vi "output.vi"(8 "error in":errorcluster, 10 "data table in":T1, 11 "Modbus Slave runtime in":refnum<class "Modbus Module runtime.lvclass">) -> (0 "error out":errorcluster, 2 "data table out":T1, 3 "Modbus Slave runtime out":refnum<class "Modbus Module runtime.lvclass">)   [LabVIEW 2015, in "Modbus Module runtime.lvclass"]
doc: "Provides an interface for writing data to a module at runtime. While this interface performs no operations, a child should provide an override which may write to any open sessions, references, or interfaces.Platypus Framework 1.0.1.65\nNI Systems Engineering - National Instruments"
uses:
  Modbus Module runtime.lvclass
  <vilib>/NI/Tag Bus/table/data table.ctl
  Modbus Module runtime.lvclass/Modbus Module runtime.ctl
  response from background process.ctl
  response enum.ctl
  message to background process.ctl
  command enum.ctl
  <vilib>/NI/Tag Bus/table/data table.lvlib
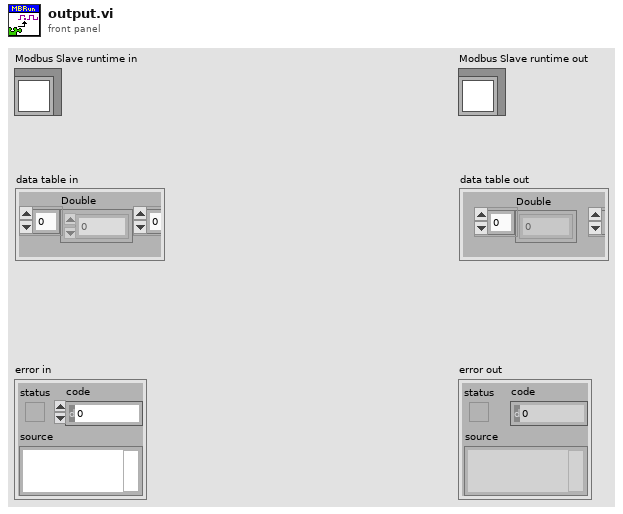
[diagram p1: front panel]
types:
  T1 = typedef "tag bus.lvlib/data table.lvlib/data table.ctl" = cluster{"Double":dbl[], "Single":sgl[], "I64":i64[], "I32":i32[], "I16":i16[], "I8":i8[], "U64":u64[], "U32":u32[], "U16":u16[], "U8":u8[], "Boolean":bool[], "String":string[], "Array of Double":cluster{"DBL Array":dbl[]}[], "Array of Single":cluster{"SGL Array":sgl[]}[], "Array of I64":cluster{"I64 Array":i64[]}[], "Array of I32":cluster{"I32 Array":i32[]}[], "Array of I16":cluster{"I16 Array":i16[]}[], "Array of I8":cluster{"I8 Array":i8[]}[], "Array of U64":cluster{"U64 Array":u64[]}[], "Array of U32":cluster{"U32 Array":u32[]}[], "Array of U16":cluster{"U16 Array":u16[]}[], "Array of U8":cluster{"U8 Array":u8[]}[], "Array of Boolean":cluster{"Boolean Array":bool[]}[], "Array of String":cluster{"String Array":string[]}[]}
  T2 = typedef "Modbus Module runtime.lvclass/response from background process.ctl" = cluster{"response enum":T3, "datapack":refnum<data-value>, "error code":i32}
  T3 = typedef "Modbus Module runtime.lvclass/response enum.ctl" = enum16{"exit", "return buffer", "error"}
  T4 = typedef "Modbus Module runtime.lvclass/command enum.ctl" = enum16{"stop", "input", "output"}
  T5 = typedef "Modbus Module runtime.lvclass/message to background process.ctl" = cluster{"command enum":T4, "datapack":refnum<data-value>}
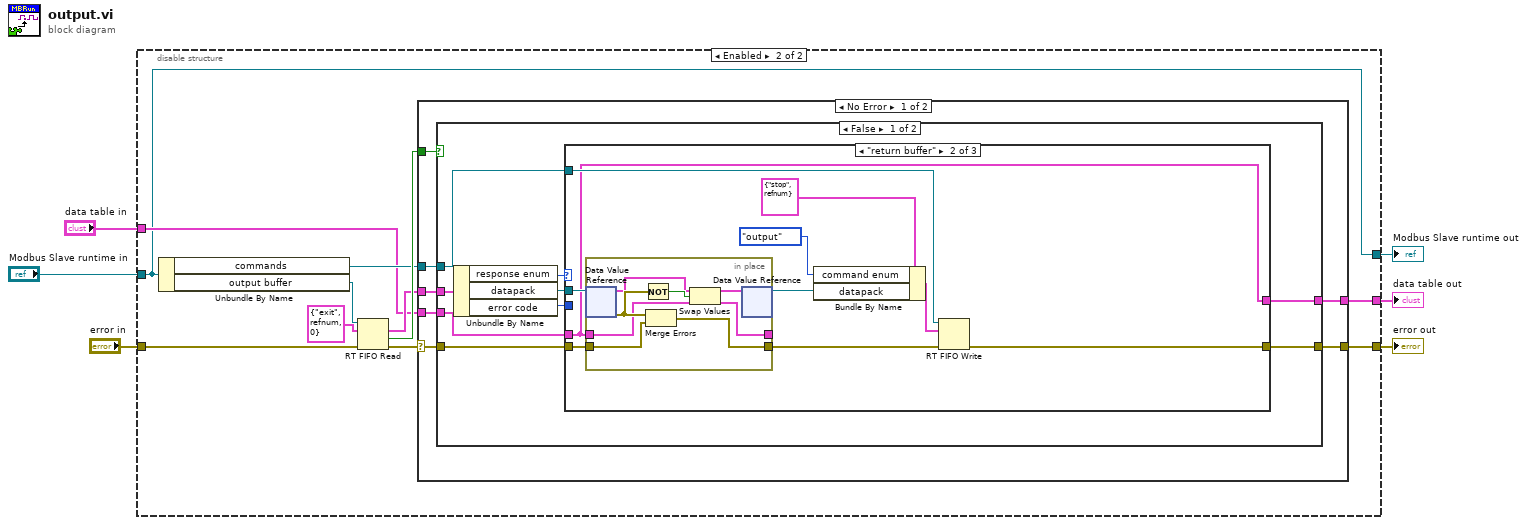
[diagram p0: block diagram]
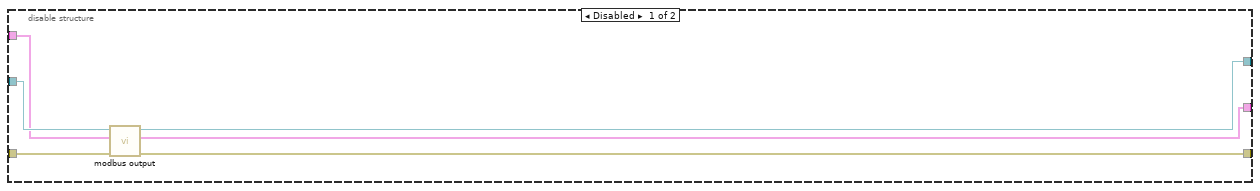
[diagram p2: hidden frame]
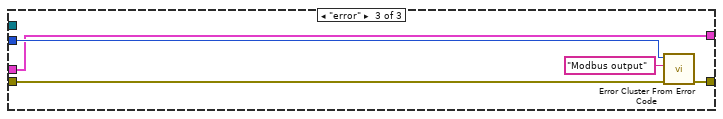
[diagram p4: hidden frame]
diagram:
  n1 = disable-structure shown="Enabled" {
    disable-tunnel: "Modbus Slave runtime in" -> [w12 w15]
    disable-tunnel: [w11 w15] -> w5
    disable-tunnel: [w10 w14] -> w4
    disable-tunnel: "data table in" -> [w9 w16]
    disable-tunnel: "error in" -> [w8 w17]
    disable-tunnel: [w7 w13] -> w1
    frame Disabled {
      n2 = call-dynamic "modbus output.vi"("error in (no error)"=w8, "data table in"=w9, "Modbus Module runtime in"=w12) -> ("error out"=w7:errorcluster, "data table out"=w10:T1, "Modbus Module runtime out"=w11:refnum<class "Modbus Module runtime.lvclass">)  [unwired: 6 in]
    }
    frame Enabled {
      n3 = Unbundle By Name(w15) -> ("commands"=w18:refnum<k33>, "output buffer"=w23:refnum<k33>)
      n4 = RT FIFO Read(0:w23, 1:T2 {"response enum"=enum."exit", "datapack"=refnum, "error code"=0} ("element"), 3:w17) -> (9:w20:T2, 10:w21:bool, 11:w19:errorcluster)  [unwired: 1 in, 2 out]
      n5 = case shown="No Error" w19 {
        selector: w19 -> [w27 w68]
        tunnel: w21 -> [w30 _]
        tunnel: w20 -> [w29 _]
        tunnel: [w28 w68] -> w13
        tunnel: w16 -> [w26 w67]
        tunnel: [w25 w67] -> w14
        tunnel: w18 -> [w24 _]
        frame No Error {
          n6 = case shown="False" w30 {
            tunnel: w29 -> [w39 _]
            tunnel: [w34 w65] -> w28
            tunnel: w27 -> [w35 w65]
            tunnel: w26 -> [w33 w66]
            tunnel: [w32 w66] -> w25
            tunnel: w24 -> [w31 _]
            frame False {
              n7 = Unbundle By Name(w39) -> ("response enum"=w37:T3, "datapack"=w38:refnum<data-value>, "error code"=w36:i32)
              n8 = case shown="\"return buffer\"" w37 {
                tunnel: w38 -> [_ w51 _]
                tunnel: w36 -> [_ _ w63]
                tunnel: w35 -> [w40 w50 w64]
                tunnel: [w40 w42 w61] -> w34
                tunnel: w33 -> [w41 w43 w60]
                tunnel: [w41 w43 w60] -> w32
                tunnel: w31 -> [_ w49 _]
                frame "exit", Default {
                }
                frame "return buffer" {
                  n9 = in-place {
                    in-place-border: w43 -> [w55]
                    in-place-border: w50 -> [w59]
                    in-place-border: [w58] -> w44
                    in-place-border: [w52] -> _
                    n10 = in-place-dvr #1(w51) -> (w54:T1, w57:errorcluster)
                    n11 = Not(x=w57) -> (.not. x?=w56:bool)
                    n12 = Merge Errors(w57, w59) -> (w58:errorcluster)
                    n13 = Swap Values(12:w54, 13:w56, 14:w55) -> (1:w53:T1, 3:w52:T1)
                    n14 = in-place-dvr #1(w53) -> (w46:refnum<data-value>)  [unwired: 1 out]
                  }
                  n15 = Bundle By Name(cluster=T5 {"command enum"=enum."stop", "datapack"=refnum} ("element"), "command enum"=command_enum."output", "datapack"=w46) -> (w45:T5)
                  n16 = RT FIFO Write(0:w49, 1:w45, 3:w44) -> (11:w42:errorcluster)  [unwired: 2 in, 3 out]
                }
                frame "error" {
                  n17 = call <vilib>:"Error Cluster From Error Code.vi"("error in (no error)"=w64, "error message (\"\")"="Modbus output" ("error message (\"\")"), "error code (0)"=w63) -> ("error out"=w61:errorcluster)  [unwired: 6 in]
                }
              }
            }
            frame True {
            }
          }
        }
        frame Error {
        }
      }
    }
  }
  "error out" <- w1
  "Modbus Slave runtime out" <- w5
  "data table out" <- w4
